vi "FuncVI-lvErrorString.vi"(5 "InstanceRef":T2, 9 "arg list":T1[](array[typedef]) {"num" format="%.2f"}) -> (0 "error out":bool, 3 "result":T1 {"num" format="%.2f"})   [LabVIEW 2021]
doc: "::: CalcExpress Toolkit :::\nCopyright (c) 2000-2026 Konstantin Shifershteyn. All rights reserved."
uses:
  cetypes.llb/CalcExpress Function Argument Info.ctl
  cetypes.llb/CalcExpress Instance RefNum.ctl
  <vilib>/Utility/error.llb/DialogType.ctl
panel:
  in  "max arg num":i32=1
  in  "min arg num":i32
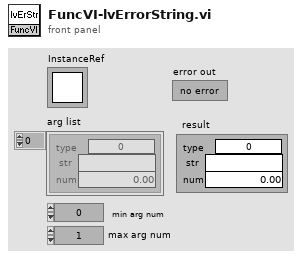
[diagram p1: front panel]
types:
  T1 = typedef "CalcExpress Function Argument Info.ctl" = cluster{"type":u32, "str":string, "num":dbl}
  T2 = typedef "CalcExpress Instance RefNum.ctl" = refnum<k1>
  T3 = enum32{"String", "DBL Number", "identifier", "1D Array of DBL", "2D Array of DBL", "CDB Number", "1D Array of CDB", "2D Array of CDB", "1D Array of String", "2D Array of String", "Unknown data type"}
  T4 = typedef "DialogType.ctl" = u16
  T5 = cluster{"data type":enum32{"String", "DBL Number", "identifier", "1D Array of DBL", "2D Array of DBL", "CDB Number", "1D Array of CDB", "2D Array of CDB", "1D Array of String", "2D Array of String", "Unknown data type"}, "data string":string, "num":dbl}
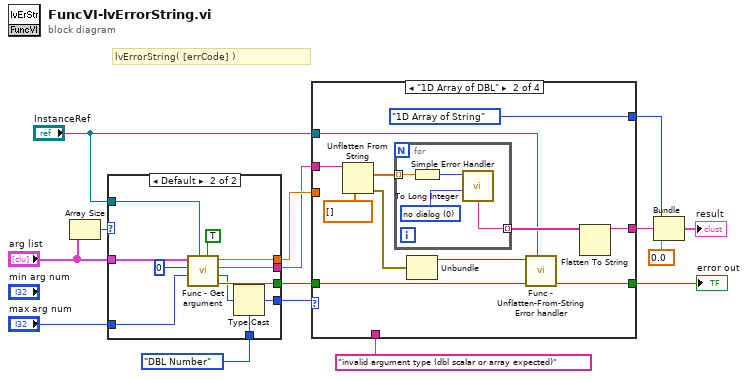
[diagram p0: block diagram]
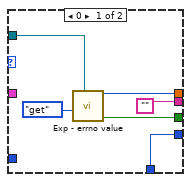
[diagram p2: hidden frame]
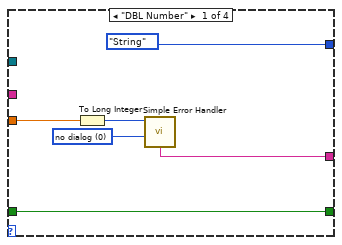
[diagram p3: hidden frame]
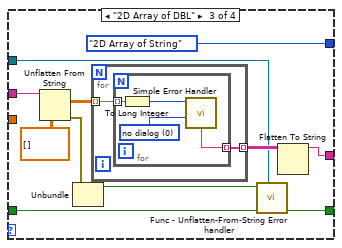
[diagram p4: hidden frame]
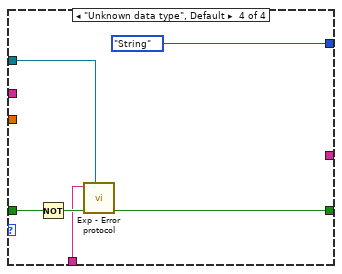
[diagram p5: hidden frame]
diagram:
  # "lvErrorString( [errCode] )"
  n1 = Array Size(array="arg list") -> (size(s)=w9:i32)
  n2 = case shown="Default" w9 {
    tunnel: "arg list" -> [_ w32]
    tunnel: [w21 w29] -> w6
    tunnel: "InstanceRef" -> [w20 w28]
    tunnel: [w18 w27] -> w5
    tunnel: ["" w26] -> w4
    tunnel: [w17 w24] -> w3
    tunnel: T3."DBL Number" ("data type") -> [w17 w23]
    tunnel: "max arg num" -> [_ w22]
    frame 0 {
      n3 = call "Exp - errno value.vi"("InstanceRef"=w20, "action"=enum32{"get", "set"}."get") -> ("error out"=w21:bool, "errno value out"=w18:i32)  [unwired: 5 in, 1 out]
    }
    frame Default {
      n4 = call "Func - Get argument.vi"("ena NonNum? (F)"=TRUE, "InstanceRef"=w28, "max arg num"=w22, "arg idx"=0, "arg list"=w32) -> ("error out"=w29:bool, "type"=w25:u32, "str"=w26:string, "num"=w27:dbl)  [unwired: 1 in]
      n5 = Type Cast(type=w23, x=w25) -> (*(type *) &x=w24:T3)
    }
  }
  n6 = case shown="\"1D Array of DBL\"" w3 {
    tunnel: [w34 w46 w61 _] -> w14
    tunnel: w5 -> [w36 _ _ _]
    tunnel: w4 -> [_ w44 w59 _]
    tunnel: w6 -> [w38 w42 w57 w76]
    tunnel: [w38 w43 w58 w74] -> w10
    tunnel: "invalid argument type (dbl scalar or array expected)" ("ErrStr") -> [_ _ _ w73]
    tunnel: "InstanceRef" -> [_ w41 w56 w72]
    tunnel: [T3."String" ("data type") T3."1D Array of String" ("data type") T3."2D Array of String" ("data type") T3."String" ("data type")] -> w12
    frame "DBL Number" {
      w33 = T4 0 items=["no dialog", "OK message", "continue or stop message", "OK message + warnings", "continue/stop + warnings"] ("type of dialog (OK msg:1)")
      n7 = To Long Integer(number=w36) -> (32bit integer=w35:i32)
      n8 = call <vilib>:"Simple Error Handler.vi"("error code (no error:0)"=w35, "type of dialog (OK msg:1)"=w33) -> ("message"=w34:string)  [unwired: 3 in, 4 out]
    }
    frame "1D Array of DBL" {
      n9 = Unflatten From String(type=dbl[] [], binary string=w44) -> (value=w48:dbl[], error out=w39:errorcluster)  [unwired: 3 in, 1 out]
      n10 = for {
        tunnel: w48 -> [w53] mode=indexing
        tunnel: [w52] -> w47 mode=indexing
        w50 = T4 0 items=["no dialog", "OK message", "continue or stop message", "OK message + warnings", "continue/stop + warnings"] ("type of dialog (OK msg:1)")
        n11 = To Long Integer(number=w53) -> (32bit integer=w51:i32)
        n12 = call <vilib>:"Simple Error Handler.vi"("error code (no error:0)"=w51, "type of dialog (OK msg:1)"=w50) -> ("message"=w52:string)  [unwired: 3 in, 4 out]
      }
      n13 = Unbundle(w39) -> ("status"=w40:bool)  [unwired: 2 out]
      n14 = call "Func - Unflatten-From-String Error handler.vi"("InstanceRef"=w41, "error in"=w42, "Unflatten Error status"=w40) -> ("error out"=w43:bool)  [unwired: 6 in]
      n15 = Flatten To String(anything=w47) -> (data string=w46:string)  [unwired: 3 in, 2 out]
    }
    frame "2D Array of DBL" {
      n16 = Unflatten From String(type=dbl[][] [], binary string=w59) -> (value=w63:dbl[][], error out=w54:errorcluster)  [unwired: 3 in, 1 out]
      n17 = Unbundle(w54) -> ("status"=w55:bool)  [unwired: 2 out]
      n18 = for {
        tunnel: w63 -> [w66] mode=indexing
        tunnel: [w65] -> w62 mode=indexing
        n19 = for {
          tunnel: w66 -> [w69] mode=indexing
          tunnel: [w70] -> w65 mode=indexing
          w67 = T4 0 items=["no dialog", "OK message", "continue or stop message", "OK message + warnings", "continue/stop + warnings"] ("type of dialog (OK msg:1)")
          n20 = To Long Integer(number=w69) -> (32bit integer=w68:i32)
          n21 = call <vilib>:"Simple Error Handler.vi"("error code (no error:0)"=w68, "type of dialog (OK msg:1)"=w67) -> ("message"=w70:string)  [unwired: 3 in, 4 out]
        }
      }
      n22 = call "Func - Unflatten-From-String Error handler.vi"("InstanceRef"=w56, "error in"=w57, "Unflatten Error status"=w55) -> ("error out"=w58:bool)  [unwired: 6 in]
      n23 = Flatten To String(anything=w62) -> (data string=w61:string)  [unwired: 3 in, 2 out]
    }
    frame "Unknown data type", Default {
      n24 = Not(x=w76) -> (.not. x?=w75:bool)
      n25 = call "Exp - Error protocol.vi"("InstanceRef"=w72, "error in"=w75, "error message in"=w73) -> ("error out"=w74:bool)  [unwired: 5 in, 1 out]
    }
  }
  "error out" <- w10
  n26 = Bundle("data type"=w12, "data string"=w14, "num"=0.0) -> (→"result":T5)  [unwired: 1 in]
